vi "Init_Elevator.vi"(8 "error in (no error)":errorcluster, 9 "AnalogOutput.lvclass":refnum<class "AnalogOutput.lvclass">, 10 "AnalogInput.lvclass":refnum<class "AnalogInput.lvclass">, 11 "Elevator in":refnum<class "Elevator.lvclass">) -> (0 "error out":errorcluster, 3 "Elevator out":refnum<class "Elevator.lvclass">)   [LabVIEW 2021, in "Elevator.lvclass"]
uses:
  Elevator.lvclass
  AnalogInput/AnalogInput.lvclass
  AnalogOutput/AnalogOutput.lvclass
  Elevator.lvclass/Elevator.ctl
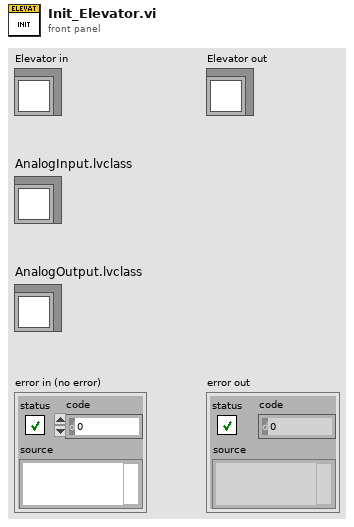
[diagram p1: front panel]
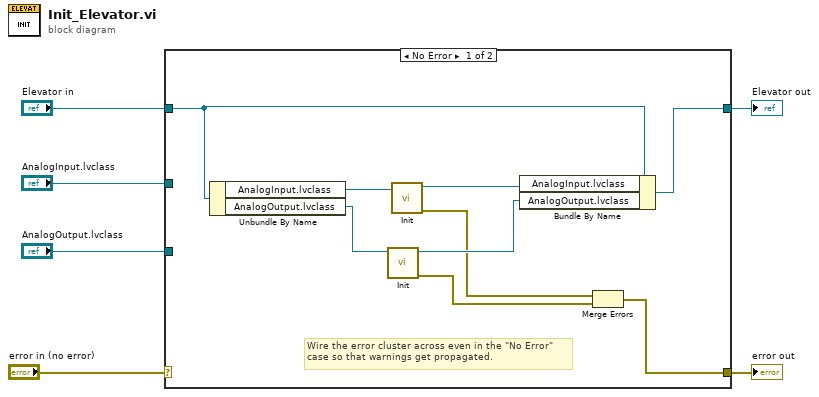
[diagram p0: block diagram]
diagram:
  n1 = case shown="No Error" "error in (no error)" {
    selector: "error in (no error)" -> [_ w17]
    tunnel: [w10 w17] -> w5
    tunnel: [w11 w16] -> w3
    tunnel: "Elevator in" -> [w9 w16]
    tunnel: "AnalogOutput.lvclass" -> [_ _]
    tunnel: "AnalogInput.lvclass" -> [_ _]
    frame No Error {
      # "Wire the error cluster across even in the \"No Error\"\ncase so that warnings get propagated."
      n2 = Unbundle By Name(w9) -> ("AnalogInput.lvclass"=w8:refnum<class "AnalogInput.lvclass">, "AnalogOutput.lvclass"=w7:refnum<class "AnalogOutput.lvclass">)
      n3 = call-dynamic "Init.vi"("AnalogOutput in"=w7) -> ("error out"=w12:errorcluster, "AnalogOutput out"=w14:refnum<class "AnalogOutput.lvclass">)  [unwired: 9 in]
      n4 = call-dynamic "Init.vi"("AnalogInput in"=w8) -> ("error out"=w13:errorcluster, "AnalogInput out"=w15:refnum<class "AnalogInput.lvclass">)  [unwired: 9 in]
      n5 = Bundle By Name(cluster=w9, "AnalogInput.lvclass"=w15, "AnalogOutput.lvclass"=w14) -> (w11:refnum<class "Elevator.lvclass">)
      n6 = Merge Errors(w13, w12) -> (w10:errorcluster)
    }
    frame Error {
    }
  }
  "error out" <- w5
  "Elevator out" <- w3
